vi "New String Handler.vi"(4 "log count limit (500)":u32=500, 6 "line count limit (500)":u32=500, 8 "auto-scroll? (T)":bool=TRUE, 9 "multi-line? (T)":bool=TRUE, 10 "formatter (format string)":refnum<class "Formatter.lvclass">, 11 "string control":refnum<vi>) -> (3 "new string handler":refnum<class "String Handler.lvclass">)   [LabVIEW 2018, in "GLog.lvlib" / "String Handler.lvclass"]
doc: "Creates a new Handler which writes log records to a string control/indicator in LabVIEW."
uses:
  String Handler.lvclass
  C:/Users/Colin/Documents/software_projects/labview/glog/src/api/extension/formatting_handler_interface/Formatting Handler.lvclass
  extension/formatter_interface/Formatter.lvclass
  String Handler.lvclass/String Handler.ctl
  extension/formatting_handler_interface/Formatting Handler.lvclass/Formatting Handler.ctl
  formatters/format_string_formatter/Format String.lvclass
  C:/Users/Colin/Documents/software_projects/labview/glog/src/api/extension/formatter_interface/Formatter.lvclass
  extension/formatting_handler_interface/Formatting Handler.lvclass
panel:
  # "Connector Pane"
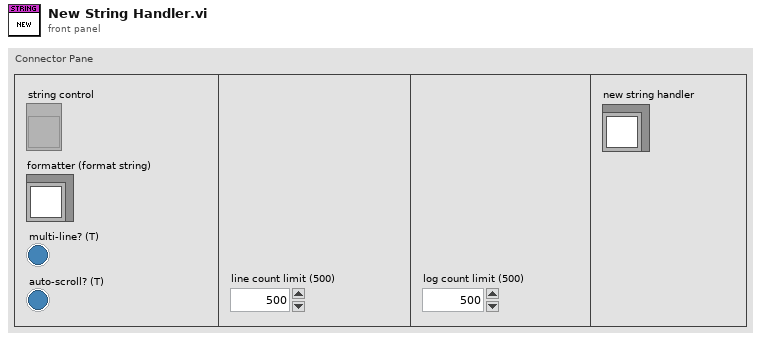
[diagram p1: front panel]
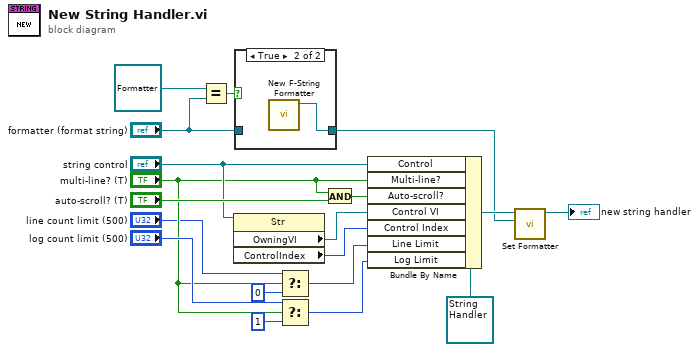
[diagram p0: block diagram]
diagram:
  n1 = Equal?(x=refnum<class "Formatter.lvclass"> refnum ("formatter (format string)"), y="formatter (format string)") -> (x = y?=w11:bool)
  n2 = property class="Str"(reference="string control") -> ("OwningVI"=w9:refnum<vi>, "ControlIndex"=w8:i32)  [unwired: 1 in, 2 out]
  n3 = case shown="True" w11 {
    tunnel: "formatter (format string)" -> [w20 _]
    tunnel: [w20 w21] -> w14
    frame False {
    }
    frame True {
      n4 = call "New F-String Formatter.vi"() -> ("new f-string formatter"=w21:refnum<class "Format String.lvclass">)  [unwired: 11 in]
    }
  }
  n5 = Select(t="line count limit (500)", s="multi-line? (T)", f=u32 0) -> (s? t:f=w3:u32)
  n6 = Select(t="log count limit (500)", s="multi-line? (T)", f=u32 1) -> (s? t:f=w6:u32)
  n7 = And(x="multi-line? (T)", y="auto-scroll? (T)") -> (x .and. y?=w16:bool)
  n8 = Bundle By Name(cluster=refnum<class "String Handler.lvclass"> refnum ("new string handler"), "Control"="string control", "Multi-line?"="multi-line? (T)", "Auto-scroll?"=w16, "Control VI"=w9, "Control Index"=w8, "Line Limit"=w3, "Log Limit"=w6) -> (w18:refnum<class "String Handler.lvclass">)
  n9 = call "Set Formatter.vi"("formatter"=w14, "handler in"=w18) -> ("handler out"=→"new string handler":refnum<class "String Handler.lvclass">)  [unwired: 9 in]
